vi "SysDef.Create.vi"(8 "error in (no error)":errorcluster, 10 "Diagnostics Configuration":T1={"Interface"="", "Baud Rate"=0, "Diagnostic Protocol"=enum."GMLAN", "Transport Protocol"=enum."ISO TP - Normal Mode", "Transmit ID"=0, "Receive ID"=0, "Transmit Extension"=0, "Receive Extension"=0, "Receive UUDT ID"=0, "Enable Stream"=TRUE, "VW TP Channel ID"=0, "Fill Frame"=FALSE, "Fill Byte"=255, "Termination"=FALSE, "LIN Cluster"="ADCS_LIN_database", "NAD"=1, "IO Mode"=0, "Max DLC"=8, "FD Baud Rate"=0, "Timeout"=0, "FD ISO Mode"=0, "DoIP Address"="", "DoIP Source Address"=3584, "DoIP Dynamic Port"=TRUE, "DoIP Version"=2} {"DoIP Version" items=["2010"=1, "2012"=2]; "DoIP Source Address" format="%.0x"; "FD ISO Mode" items=["ISO", "Non ISO", "ISO Legacy"]; "IO Mode" items=["CAN 2.0", "CAN FD", "CAN FD+BRS"]; "Fill Byte" format="%.0x"; "VW TP Channel ID" format="%.0x"; "Receive UUDT ID" format="%.0x"; "Receive Extension" format="%.0x"; "Transmit Extension" format="%.0x"; "Receive ID" format="%.0x"; "Transmit ID" format="%.0x"}, 11 "Device Item Ref in":T5 format="%.0x") -> (0 "error out":errorcluster, 3 "Device Item Ref out":T5 format="%.0x")   [LabVIEW 2024, in "Diagnostics Addon System Explorer.lvlib"]
uses:
  Diagnostics Addon System Explorer.lvlib
  Types/FG.Action.ctl
  <vilib>/NI VeriStand/Custom Device API/Custom Device Channel.ctl
  <vilib>/NI VeriStand/Custom Device API/Custom Device API.lvlib
  <vilib>/NI VeriStand/Custom Device API/Custom Device Channel Type.ctl
  Addon Shared/SubVIs/Constants.vi
  Addon Shared/Diagnostics Addon Shared.lvlib
  <vilib>/NI/NI VeriStand Advanced SysDef API/SysDef API/Advanced System Definition.lvlib
  Addon Shared/Types/Type.ctl
  Addon Shared/Types/Command.New.ctl
  <userlib>/_OpenG.lib/lvdata/lvdata.llb/openg_variant.lvlib
  <vilib>/NI VeriStand/Custom Device API/Custom Device Item Ref.ctl
  Addon Shared/Types/CAN.ctl
  Addon Shared/Types/Protocol.ctl
  Addon Shared/Types/CAN.Interface.ctl
  Addon Shared/Types/Transport.ctl
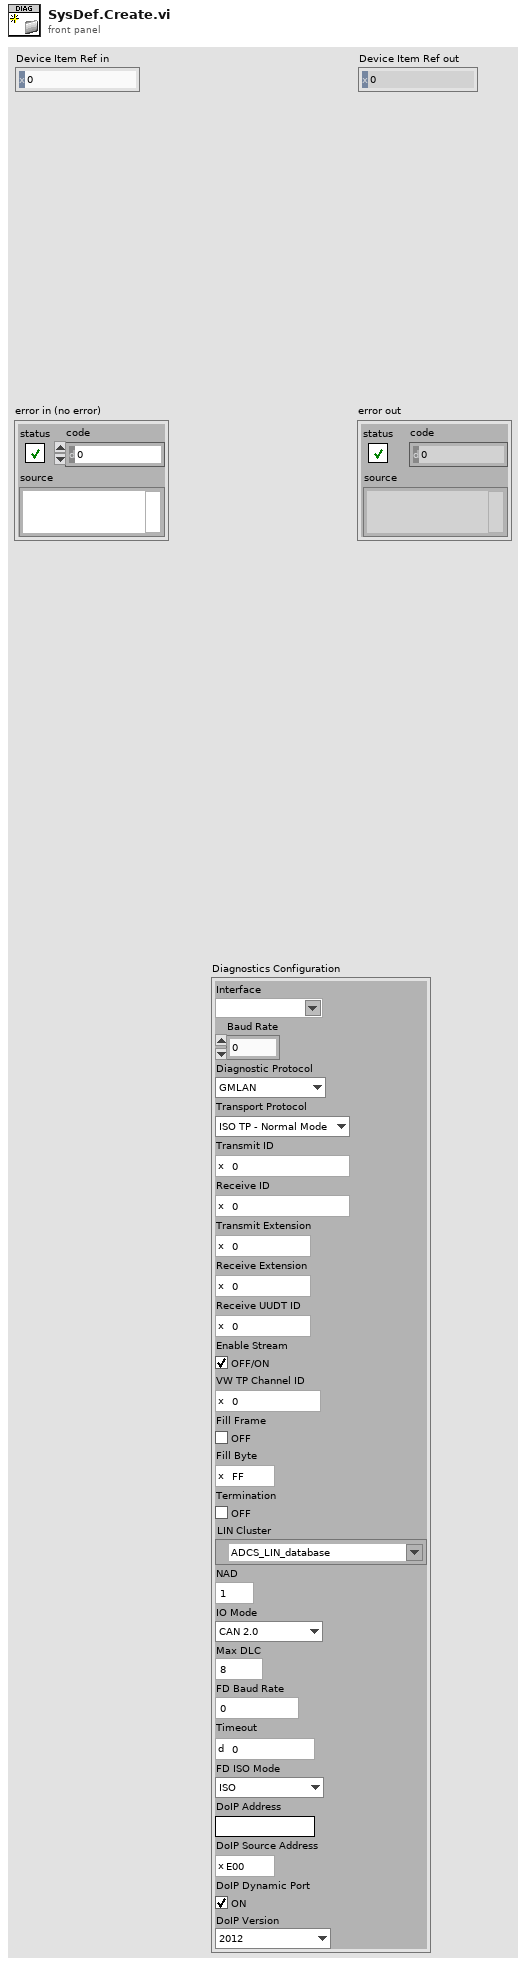
[diagram p1: front panel]
types:
  T1 = typedef "Diagnostics Addon Shared.lvlib/CAN.ctl" = cluster{"Interface":T2, "Baud Rate":u64, "Diagnostic Protocol":T3, "Transport Protocol":T4, "Transmit ID":u32, "Receive ID":u32, "Transmit Extension":u8, "Receive Extension":u8, "Receive UUDT ID":u32, "Enable Stream":bool, "VW TP Channel ID":u32, "Fill Frame":bool, "Fill Byte":u8, "Termination":bool, "LIN Cluster":refnum<k21>, "NAD":u8, "IO Mode":u32, "Max DLC":u16, "FD Baud Rate":u64, "Timeout":u32, "FD ISO Mode":u32, "DoIP Address":string, "DoIP Source Address":u16, "DoIP Dynamic Port":bool, "DoIP Version":u16}
  T2 = typedef "Diagnostics Addon Shared.lvlib/CAN.Interface.ctl" = string
  T3 = typedef "Diagnostics Addon Shared.lvlib/Protocol.ctl" = enum16{"GMLAN", "KWP-2000", "UDS", "User-Defined"}
  T4 = typedef "Diagnostics Addon Shared.lvlib/Transport.ctl" = enum16{"ISO TP - Normal Mode", "ISO TP - Mixed Mode", "VW TP 2.0", "Diagnostics on IP", "ISO TP LIN"}
  T5 = typedef "Custom Device API.lvlib/Custom Device Item Ref.ctl" = u64
  T6 = typedef "Custom Device API.lvlib/Custom Device Channel.ctl" = cluster{"Type":T7, "Units":string, "Default Value":dbl, "Faultable":bool, "Scalable":bool}
  T7 = typedef "Custom Device API.lvlib/Custom Device Channel Type.ctl" = enum16{"Input", "Output"}
  T8 = typedef "Diagnostics Addon Shared.lvlib/Command.New.ctl" = enum8{"None", "Clear Status Channels", "Read All DIDs", "Read All PIDs", "Configure and Start DPIDs", "Stop DPIDs"}
  T9 = typedef "Diagnostics Addon System Explorer.lvlib/FG.Action.ctl" = enum16{"Get", "Set"}
  T10 = typedef "Diagnostics Addon Shared.lvlib/Type.ctl" = enum16{"DID", "CDID", "PID", "CPID", "Read Memory", "Write Memory", "IO Control", "Routine Start", "Routine Request", "Routine Stop", "User Defined", "DTC Control", "Clear DTCs", "Read DTCs", "Start DTCs", "DTC Change Count", "Tester Present", "Unlock ECU", "Reset ECU", "Diag Session Control", "Communication Control", "DPID Control", "Poll Control", "Diag Comm Port Control"}
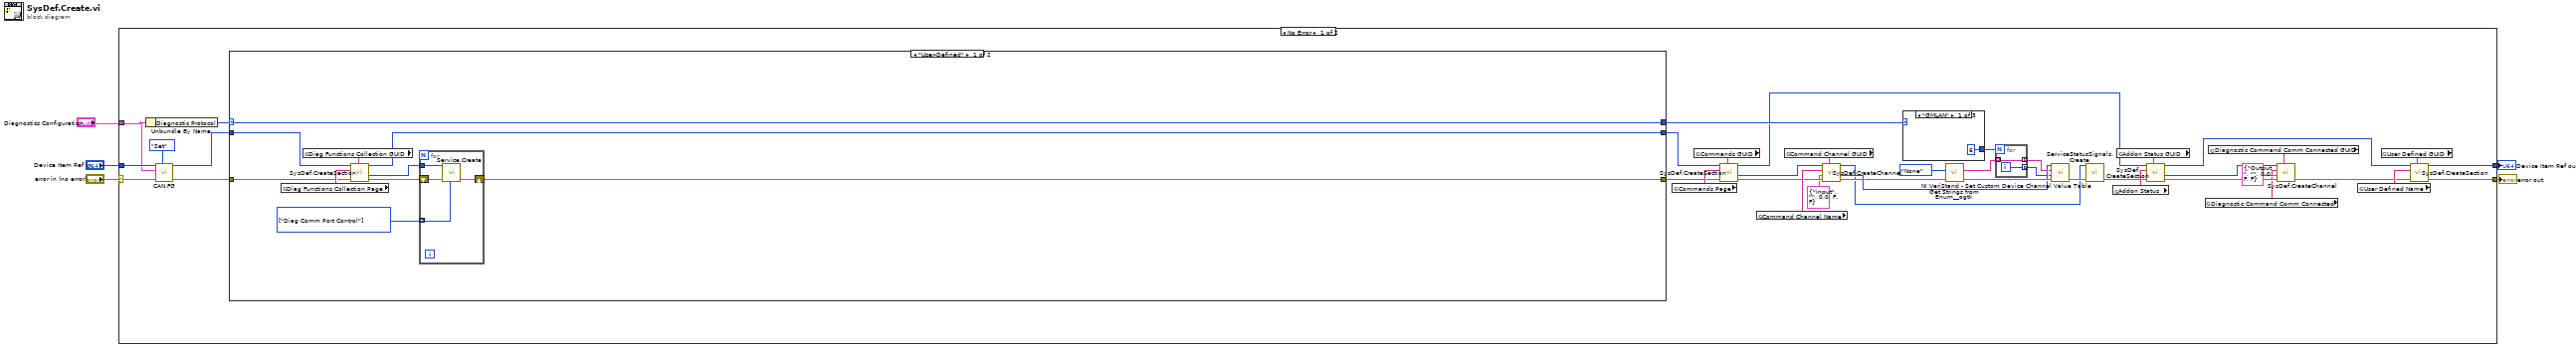
[diagram p0: block diagram]
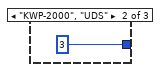
[diagram p2: hidden frame]
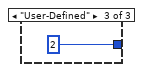
[diagram p3: hidden frame]
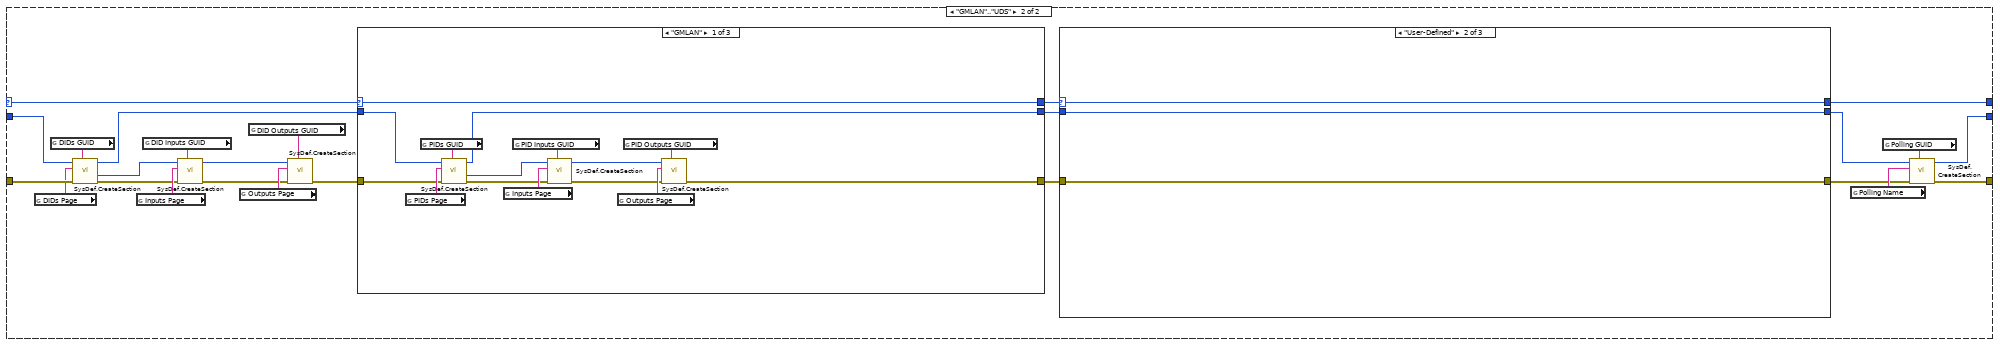
[diagram p4: hidden frame]
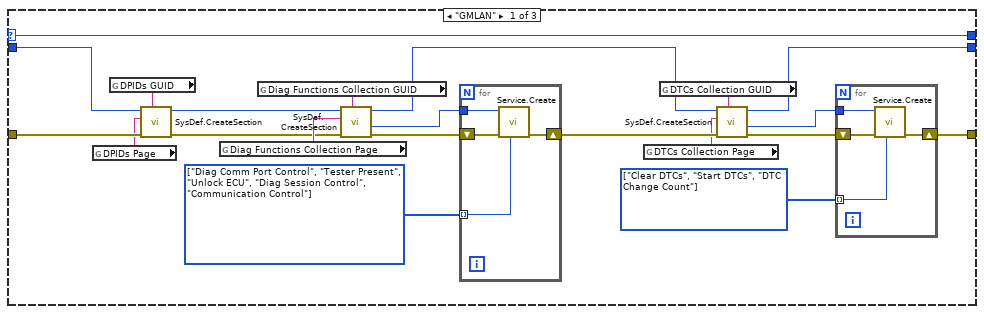
[diagram p5: hidden frame]
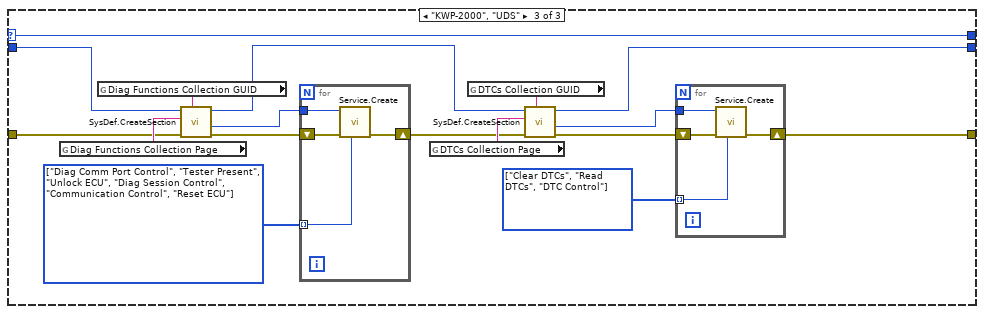
[diagram p6: hidden frame]
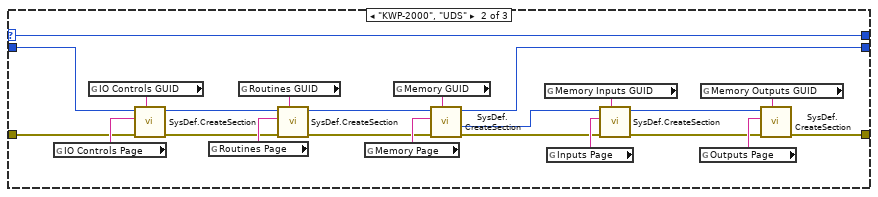
[diagram p7: hidden frame]
diagram:
  n1 = case shown="No Error" "error in (no error)" {
    selector: "error in (no error)" -> [w41 w191]
    tunnel: [w32 w191] -> w4
    tunnel: "Device Item Ref in" -> [w40 w190]
    tunnel: [w33 w190] -> w2
    tunnel: "Diagnostics Configuration" -> [w36 _]
    frame No Error {
      n2 = Unbundle By Name(w36) -> ("Diagnostic Protocol"=w37:T3)
      n3 = call "CAN.FG.vi"("Action"=FG.Action."Set", "error in (no error)"=w41, "Diagnostics Basic Configuration"=w36, "Device Item Ref in"=w40) -> ("error out"=w39:errorcluster, "Device Item Ref out"=w38:T5)  [unwired: 5 in, 1 out]
      n4 = case shown="\"User-Defined\"" w37 {
        selector: w37 -> [w62 w75]
        tunnel: w39 -> [w56 w91]
        tunnel: w38 -> [w54 w90]
        tunnel: [w55 w77] -> w20
        tunnel: [w53 w68] -> w21
        tunnel: [w62 w67] -> w22
        frame "User-Defined" {
          w57 = T10[] [enum."Diag Comm Port Control"] items=["DID", "CDID", "PID", "CPID", "Read Memory", "Write Memory", "IO Control", "Routine Start", "Routine Request", "Routine Stop", "User Defined", "DTC Control", "Clear DTCs", "Read DTCs", "Start DTCs", "DTC Change Count", "Tester Present", "Unlock ECU", "Reset ECU", "Diag Session Control", "Communication Control", "DPID Control", "Poll Control", "Diag Comm Port Control"]
          n5 = global read "Constants.vi" "Diag Functions Collection Page"() -> (w58:string)
          n6 = global read "Constants.vi" "Diag Functions Collection GUID"() -> (w59:string)
          n7 = call <vilib>:"SysDef.CreateSection.vi"("GUID"=w59, "error in (no error)"=w56, "Name"=w58, "nodeID"=w54) -> ("error out"=w60:errorcluster, "New NodeID"=w61:u64, "nodeID out"=w55:u64)  [unwired: 4 in, 1 out]
          n8 = for {
            tunnel: w61 -> [w65]
            shift-right: [w64] -> w53
            shift-left: w60 -> [w66]
            tunnel: w57 -> [w63] mode=indexing
            n9 = call "Service.Create.vi"("Type"=w63, "error in (no error)"=w66, "Section Ptr"=w65) -> ("error out"=w64:errorcluster)  [unwired: 7 in, 1 out]
          }
        }
        frame "GMLAN".."UDS" {
          n10 = global read "Constants.vi" "DIDs Page"() -> (w89:string)
          n11 = global read "Constants.vi" "DIDs GUID"() -> (w88:string)
          n12 = call <vilib>:"SysDef.CreateSection.vi"("GUID"=w88, "error in (no error)"=w91, "Name"=w89, "nodeID"=w90) -> ("error out"=w85:errorcluster, "New NodeID"=w84:u64, "nodeID out"=w74:u64)  [unwired: 4 in, 1 out]
          n13 = global read "Constants.vi" "Inputs Page"() -> (w86:string)
          n14 = global read "Constants.vi" "DID Inputs GUID"() -> (w87:string)
          n15 = call <vilib>:"SysDef.CreateSection.vi"("GUID"=w87, "error in (no error)"=w85, "Name"=w86, "nodeID"=w84) -> ("error out"=w78:errorcluster, "nodeID out"=w81:u64)  [unwired: 4 in, 2 out]
          n16 = global read "Constants.vi" "Outputs Page"() -> (w82:string)
          n17 = global read "Constants.vi" "DID Outputs GUID"() -> (w83:string)
          n18 = call <vilib>:"SysDef.CreateSection.vi"("GUID"=w83, "error in (no error)"=w78, "Name"=w82, "nodeID"=w81) -> ("error out"=w76:errorcluster)  [unwired: 4 in, 3 out]
          n19 = case shown="\"GMLAN\"" w75 {
            selector: w75 -> [w155 w164 w187]
            tunnel: w76 -> [w157 w169 w189]
            tunnel: w74 -> [w156 w182 w188]
            tunnel: [w154 w177 w188] -> w70
            tunnel: [w149 w165 w189] -> w72
            tunnel: [w155 w164 w187] -> w71
            frame "GMLAN" {
              n20 = global read "Constants.vi" "PIDs Page"() -> (w159:string)
              n21 = global read "Constants.vi" "PIDs GUID"() -> (w158:string)
              n22 = call <vilib>:"SysDef.CreateSection.vi"("GUID"=w158, "error in (no error)"=w157, "Name"=w159, "nodeID"=w156) -> ("error out"=w153:errorcluster, "New NodeID"=w152:u64, "nodeID out"=w154:u64)  [unwired: 4 in, 1 out]
              n23 = global read "Constants.vi" "Inputs Page"() -> (w161:string)
              n24 = global read "Constants.vi" "PID Inputs GUID"() -> (w160:string)
              n25 = call <vilib>:"SysDef.CreateSection.vi"("GUID"=w160, "error in (no error)"=w153, "Name"=w161, "nodeID"=w152) -> ("error out"=w151:errorcluster, "nodeID out"=w150:u64)  [unwired: 4 in, 2 out]
              n26 = global read "Constants.vi" "Outputs Page"() -> (w163:string)
              n27 = global read "Constants.vi" "PID Outputs GUID"() -> (w162:string)
              n28 = call <vilib>:"SysDef.CreateSection.vi"("GUID"=w162, "error in (no error)"=w151, "Name"=w163, "nodeID"=w150) -> ("error out"=w149:errorcluster)  [unwired: 4 in, 3 out]
            }
            frame "KWP-2000", "UDS" {
              n29 = global read "Constants.vi" "IO Controls Page"() -> (w183:string)
              n30 = global read "Constants.vi" "IO Controls GUID"() -> (w184:string)
              n31 = call <vilib>:"SysDef.CreateSection.vi"("GUID"=w184, "error in (no error)"=w169, "Name"=w183, "nodeID"=w182) -> ("error out"=w168:errorcluster, "nodeID out"=w181:u64)  [unwired: 4 in, 2 out]
              n32 = global read "Constants.vi" "Routines Page"() -> (w186:string)
              n33 = global read "Constants.vi" "Routines GUID"() -> (w185:string)
              n34 = call <vilib>:"SysDef.CreateSection.vi"("GUID"=w185, "error in (no error)"=w168, "Name"=w186, "nodeID"=w181) -> ("error out"=w167:errorcluster, "nodeID out"=w178:u64)  [unwired: 4 in, 2 out]
              n35 = global read "Constants.vi" "Memory Page"() -> (w179:string)
              n36 = global read "Constants.vi" "Memory GUID"() -> (w180:string)
              n37 = call <vilib>:"SysDef.CreateSection.vi"("GUID"=w180, "error in (no error)"=w167, "Name"=w179, "nodeID"=w178) -> ("error out"=w171:errorcluster, "New NodeID"=w170:u64, "nodeID out"=w177:u64)  [unwired: 4 in, 1 out]
              n38 = global read "Constants.vi" "Memory Inputs GUID"() -> (w176:string)
              n39 = global read "Constants.vi" "Inputs Page"() -> (w175:string)
              n40 = call <vilib>:"SysDef.CreateSection.vi"("GUID"=w176, "error in (no error)"=w171, "Name"=w175, "nodeID"=w170) -> ("error out"=w166:errorcluster, "nodeID out"=w174:u64)  [unwired: 4 in, 2 out]
              n41 = global read "Constants.vi" "Outputs Page"() -> (w173:string)
              n42 = global read "Constants.vi" "Memory Outputs GUID"() -> (w172:string)
              n43 = call <vilib>:"SysDef.CreateSection.vi"("GUID"=w172, "error in (no error)"=w166, "Name"=w173, "nodeID"=w174) -> ("error out"=w165:errorcluster)  [unwired: 4 in, 3 out]
            }
            frame "User-Defined" {
            }
          }
          n44 = case shown="\"User-Defined\"" w71 {
            selector: w71 -> [w92 w123 w124]
            tunnel: [w111 w121 w126] -> w69
            tunnel: [w112 w122 w127] -> w73
            tunnel: w72 -> [w103 w122 w128]
            tunnel: w70 -> [w102 w121 w125]
            tunnel: [w92 w123 w124] -> w67
            frame "GMLAN" {
              w97 = T10[] [enum."Clear DTCs", enum."Start DTCs", enum."DTC Change Count"] items=["DID", "CDID", "PID", "CPID", "Read Memory", "Write Memory", "IO Control", "Routine Start", "Routine Request", "Routine Stop", "User Defined", "DTC Control", "Clear DTCs", "Read DTCs", "Start DTCs", "DTC Change Count", "Tester Present", "Unlock ECU", "Reset ECU", "Diag Session Control", "Communication Control", "DPID Control", "Poll Control", "Diag Comm Port Control"]
              w98 = T10[] [enum."Diag Comm Port Control", enum."Tester Present", enum."Unlock ECU", enum."Diag Session Control", enum."Communication Control"] items=["DID", "CDID", "PID", "CPID", "Read Memory", "Write Memory", "IO Control", "Routine Start", "Routine Request", "Routine Stop", "User Defined", "DTC Control", "Clear DTCs", "Read DTCs", "Start DTCs", "DTC Change Count", "Tester Present", "Unlock ECU", "Reset ECU", "Diag Session Control", "Communication Control", "DPID Control", "Poll Control", "Diag Comm Port Control"]
              n45 = global read "Constants.vi" "DPIDs Page"() -> (w94:string)
              n46 = global read "Constants.vi" "DPIDs GUID"() -> (w93:string)
              n47 = call <vilib>:"SysDef.CreateSection.vi"("GUID"=w93, "error in (no error)"=w103, "Name"=w94, "nodeID"=w102) -> ("error out"=w95:errorcluster, "nodeID out"=w100:u64)  [unwired: 4 in, 2 out]
              n48 = global read "Constants.vi" "Diag Functions Collection Page"() -> (w104:string)
              n49 = global read "Constants.vi" "Diag Functions Collection GUID"() -> (w105:string)
              n50 = call <vilib>:"SysDef.CreateSection.vi"("GUID"=w105, "error in (no error)"=w95, "Name"=w104, "nodeID"=w100) -> ("error out"=w106:errorcluster, "New NodeID"=w107:u64, "nodeID out"=w101:u64)  [unwired: 4 in, 1 out]
              n51 = for {
                tunnel: w107 -> [w115]
                shift-right: [w114] -> w99
                shift-left: w106 -> [w116]
                tunnel: w98 -> [w113] mode=indexing
                n52 = call "Service.Create.vi"("Type"=w113, "error in (no error)"=w116, "Section Ptr"=w115) -> ("error out"=w114:errorcluster)  [unwired: 7 in, 1 out]
              }
              n53 = global read "Constants.vi" "DTCs Collection Page"() -> (w96:string)
              n54 = global read "Constants.vi" "DTCs Collection GUID"() -> (w110:string)
              n55 = call <vilib>:"SysDef.CreateSection.vi"("GUID"=w110, "error in (no error)"=w99, "Name"=w96, "nodeID"=w101) -> ("error out"=w109:errorcluster, "New NodeID"=w108:u64, "nodeID out"=w111:u64)  [unwired: 4 in, 1 out]
              n56 = for {
                tunnel: w108 -> [w119]
                shift-right: [w118] -> w112
                shift-left: w109 -> [w120]
                tunnel: w97 -> [w117] mode=indexing
                n57 = call "Service.Create.vi"("Type"=w117, "error in (no error)"=w120, "Section Ptr"=w119) -> ("error out"=w118:errorcluster)  [unwired: 7 in, 1 out]
              }
            }
            frame "User-Defined" {
            }
            frame "KWP-2000", "UDS" {
              w129 = T10[] [enum."Clear DTCs", enum."Read DTCs", enum."DTC Control"] items=["DID", "CDID", "PID", "CPID", "Read Memory", "Write Memory", "IO Control", "Routine Start", "Routine Request", "Routine Stop", "User Defined", "DTC Control", "Clear DTCs", "Read DTCs", "Start DTCs", "DTC Change Count", "Tester Present", "Unlock ECU", "Reset ECU", "Diag Session Control", "Communication Control", "DPID Control", "Poll Control", "Diag Comm Port Control"]
              w130 = T10[] [enum."Diag Comm Port Control", enum."Tester Present", enum."Unlock ECU", enum."Diag Session Control", enum."Communication Control", enum."Reset ECU"] items=["DID", "CDID", "PID", "CPID", "Read Memory", "Write Memory", "IO Control", "Routine Start", "Routine Request", "Routine Stop", "User Defined", "DTC Control", "Clear DTCs", "Read DTCs", "Start DTCs", "DTC Change Count", "Tester Present", "Unlock ECU", "Reset ECU", "Diag Session Control", "Communication Control", "DPID Control", "Poll Control", "Diag Comm Port Control"]
              n58 = global read "Constants.vi" "Diag Functions Collection Page"() -> (w133:string)
              n59 = global read "Constants.vi" "Diag Functions Collection GUID"() -> (w134:string)
              n60 = call <vilib>:"SysDef.CreateSection.vi"("GUID"=w134, "error in (no error)"=w128, "Name"=w133, "nodeID"=w125) -> ("error out"=w135:errorcluster, "New NodeID"=w136:u64, "nodeID out"=w132:u64)  [unwired: 4 in, 1 out]
              n61 = for {
                tunnel: w136 -> [w143]
                shift-right: [w142] -> w131
                shift-left: w135 -> [w144]
                tunnel: w130 -> [w141] mode=indexing
                n62 = call "Service.Create.vi"("Type"=w141, "error in (no error)"=w144, "Section Ptr"=w143) -> ("error out"=w142:errorcluster)  [unwired: 7 in, 1 out]
              }
              n63 = global read "Constants.vi" "DTCs Collection Page"() -> (w140:string)
              n64 = global read "Constants.vi" "DTCs Collection GUID"() -> (w139:string)
              n65 = call <vilib>:"SysDef.CreateSection.vi"("GUID"=w139, "error in (no error)"=w131, "Name"=w140, "nodeID"=w132) -> ("error out"=w138:errorcluster, "New NodeID"=w137:u64, "nodeID out"=w126:u64)  [unwired: 4 in, 1 out]
              n66 = for {
                tunnel: w137 -> [w147]
                shift-right: [w146] -> w127
                shift-left: w138 -> [w148]
                tunnel: w129 -> [w145] mode=indexing
                n67 = call "Service.Create.vi"("Type"=w145, "error in (no error)"=w148, "Section Ptr"=w147) -> ("error out"=w146:errorcluster)  [unwired: 7 in, 1 out]
              }
            }
          }
          n68 = global read "Constants.vi" "Polling Name"() -> (w80:string)
          n69 = global read "Constants.vi" "Polling GUID"() -> (w79:string)
          n70 = call <vilib>:"SysDef.CreateSection.vi"("GUID"=w79, "error in (no error)"=w73, "Name"=w80, "nodeID"=w69) -> ("error out"=w68:errorcluster, "nodeID out"=w77:u64)  [unwired: 4 in, 2 out]
        }
      }
      n71 = global read "Constants.vi" "Commands Page"() -> (w47:string)
      n72 = global read "Constants.vi" "Commands GUID"() -> (w46:string)
      n73 = call <vilib>:"SysDef.CreateSection.vi"("GUID"=w46, "error in (no error)"=w21, "Name"=w47, "nodeID"=w20) -> ("error out"=w35:errorcluster, "New NodeID"=w34:u64, "nodeID out"=w13:u64)  [unwired: 4 in, 1 out]
      n74 = global read "Constants.vi" "Command Channel Name"() -> (w42:string)
      n75 = global read "Constants.vi" "Command Channel GUID"() -> (w30:string)
      n76 = call <vilib>:"SysDef.CreateChannel.vi"("GUID"=w30, "error in (no error)"=w35, "Channel"=T6 {"Type"=enum."Input", "Units"="", "Default Value"=0.0, "Faultable"=FALSE, "Scalable"=FALSE}, "Name"=w42, "nodeID"=w34) -> ("error out"=w18:errorcluster, "New NodeID"=w27:u64, "nodeID out"=w17:u64)  [unwired: 3 in, 1 out]
      n77 = case shown="\"GMLAN\"" w22 {
        tunnel: [6 3 2] -> w23
        frame "GMLAN" {
        }
        frame "KWP-2000", "UDS" {
        }
        frame "User-Defined" {
        }
      }
      n78 = call <userlib>:"Get Strings from Enum__ogtk.vi"("error in (no error)"=w18, "Enum"=Command.New."None") -> ("error out"=w28:errorcluster, "Enum Strings"=w26:string[])  [unwired: 6 in, 2 out]
      n79 = for {
        N: w23 -> [_]
        tunnel: w26 -> [w51] mode=indexing
        tunnel: [w52] -> w24 mode=indexing
        tunnel: [w51] -> w25 mode=indexing
        i -> [w52]
      }
      n80 = call <vilib>:"NI VeriStand - Set Custom Device Channel Value Table.vi"("error in (no error)"=w28, "Values"=w24, "Names"=w25, "Channel Ref in"=w27) -> ("error out"=w19:errorcluster)  [unwired: 6 in, 1 out]
      n81 = call "ServiceStatusSignals.Create.vi"("error in (no error)"=w19, "nodeID in"=w17) -> ("error out"=w14:errorcluster)  [unwired: 8 in, 1 out]
      n82 = global read "Constants.vi" "Addon Status"() -> (w16:string)
      n83 = global read "Constants.vi" "Addon Status GUID"() -> (w15:string)
      n84 = call <vilib>:"SysDef.CreateSection.vi"("GUID"=w15, "error in (no error)"=w14, "Name"=w16, "nodeID"=w13) -> ("error out"=w9:errorcluster, "New NodeID"=w10:u64, "nodeID out"=w6:u64)  [unwired: 4 in, 1 out]
      n85 = global read "Constants.vi" "Diagnostic Command Comm Connected"() -> (w7:string)
      n86 = global read "Constants.vi" "Diagnostic Command Comm Connected GUID"() -> (w11:string)
      n87 = call <vilib>:"SysDef.CreateChannel.vi"("GUID"=w11, "error in (no error)"=w9, "Channel"=T6 {"Type"=enum."Output", "Units"="", "Default Value"=0.0, "Faultable"=FALSE, "Scalable"=FALSE}, "Name"=w7, "nodeID"=w10) -> ("error out"=w8:errorcluster)  [unwired: 3 in, 3 out]
      n88 = global read "Constants.vi" "User Defined Name"() -> (w43:string)
      n89 = global read "Constants.vi" "User Defined GUID"() -> (w44:string)
      n90 = call <vilib>:"SysDef.CreateSection.vi"("GUID"=w44, "error in (no error)"=w8, "Name"=w43, "nodeID"=w6) -> ("error out"=w32:errorcluster, "nodeID out"=w33:u64)  [unwired: 4 in, 2 out]
    }
    frame Error {
    }
  }
  "error out" <- w4
  "Device Item Ref out" <- w2
